vi "Stream LLP Packets to Disk.vi"(0 "fpga interface in":refnum<k20>, 1 "bytes acquired indicator ref":refnum<vi>, 5 "serial input channel":string, 7 "base packet file path":path, 9 "fetch size (elements)":u32=40960, 11 "error in (no error)":errorcluster, 12 "fetch timeout (s)":dbl=1.0, 13 "log to disk":bool=TRUE) -> (4 "fpga interface out":refnum<k20>, 6 "file path out":path, 8 "acquisition error":bool, 15 "error out":errorcluster)   [LabVIEW 2023, in "GettingStarted_Acq_148X_Host.lvlib"]
uses:
  GettingStarted_Acq_148X_Host.lvlib
  Types/148x_Acq_FPGA_Reference.ctl
  0829f115-c11d-4785-86b3-38f743f517d6.vi
  <vilib>/rvi/errors/niLvFpgaAdjustHostInterfaceError.vi
  <vilib>/rvi/interface/nirviMethod/nirviMethod.xnode
  <vilib>/rvi/interface/nirviReadWriteControl/nirviReadWriteControl.xnode
  <vilib>/FPGAPlugInAG/Dynamic/niLvFpga_AcquireReadRegionFifo_Dynamic.vi
  <vilib>/rvi/errors/niLvFpgaMergeErrorWithErrorCode.vi
  <instrlib>/FlexRIO/Automotive Vision Utility/v1/Host/Automotive Vision Utility.lvlib
  Common/GettingStarted_Common_148X_Host.lvlib
  NiFpgaLv.dll
  <vilib>/rvi/interface/Simulation/niFpgaSimulationCallBeginRW.vi
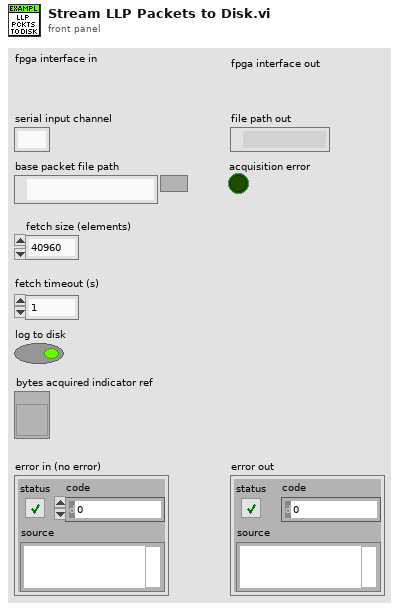
[diagram p1: front panel]
types:
  T1 = typedef "Automotive Vision Utility.lvlib/Serial Channel Type.ctl" = enum16{"Serial Input Channel", "Serial Output Channel", "Unknown Channel Type"}
  T2 = typedef "GettingStarted_Acq_148X_Host.lvlib/148x_Acq_FPGA_Reference.ctl" = refnum<k20>
  T3 = enum16{"open", "open or create", "create or replace", "create", "open (read-only)"}
  T4 = cluster{"acq state":enum8{"Idle", "Wait for First Packet Header", "Acquire", "Wait for Last Packet Header", "Wait for End of Last Packet"}, "stop timed out":bool, "bad packet header":bool, "bad packet payload":bool, "bad packet size":bool, "dram status":cluster{"bytes written":u64, "bytes read":u64, "overflow":bool, "partition full":bool, "last byte flushed":bool}}[]
  T5 = cluster{"acq state":enum8{"Idle", "Wait for First Packet Header", "Acquire", "Wait for Last Packet Header", "Wait for End of Last Packet"}, "stop timed out":bool, "bad packet header":bool, "bad packet payload":bool, "bad packet size":bool, "dram status":cluster{"bytes written":u64, "bytes read":u64, "overflow":bool, "partition full":bool, "last byte flushed":bool}}
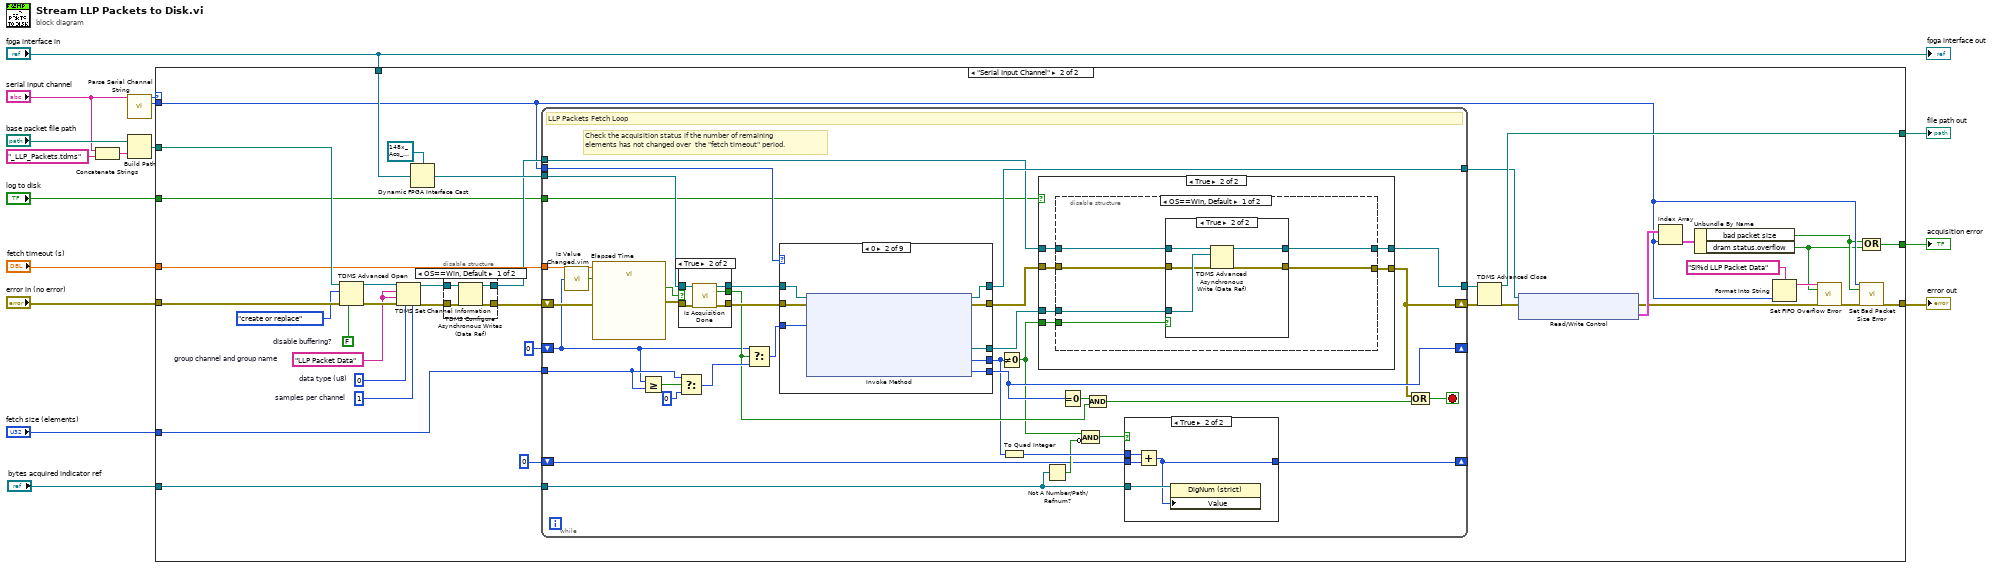
[diagram p0: block diagram]
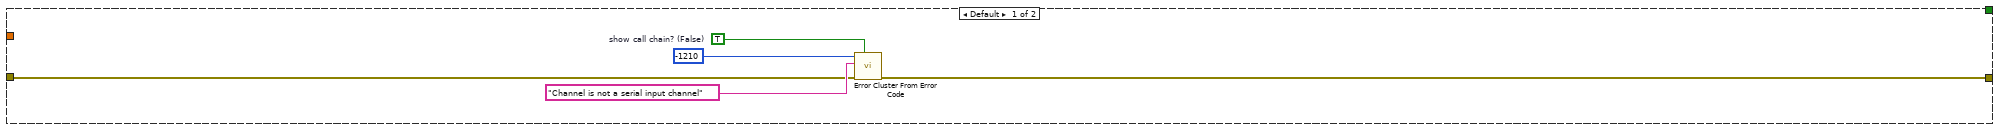
[diagram p2: hidden frame]
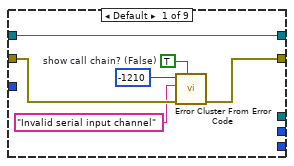
[diagram p6: hidden frame]
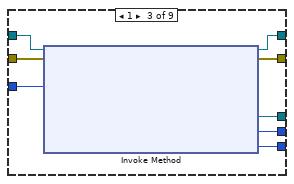
[diagram p7: hidden frame]
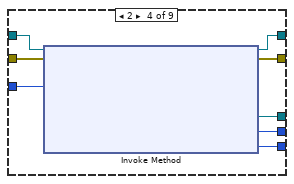
[diagram p8: hidden frame]
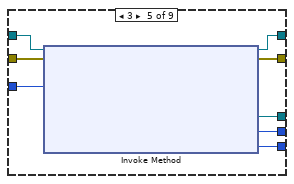
[diagram p9: hidden frame]
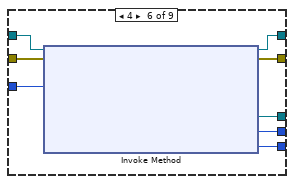
[diagram p10: hidden frame]
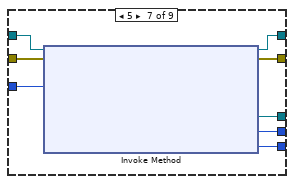
[diagram p11: hidden frame]
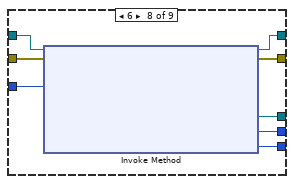
[diagram p12: hidden frame]
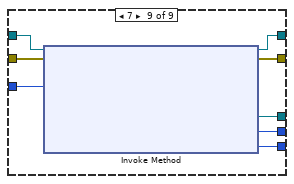
[diagram p13: hidden frame]
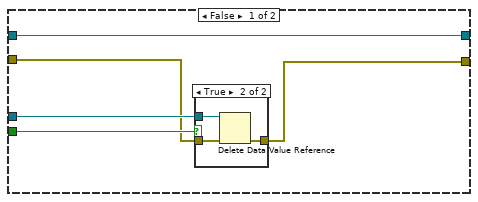
[diagram p14: hidden frame]
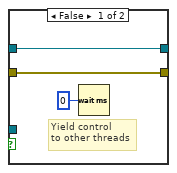
[diagram p16: hidden frame]
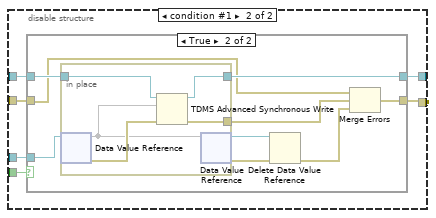
[diagram p17: hidden frame]
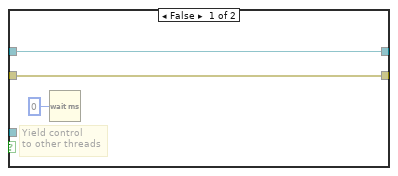
[diagram p18: hidden frame]
diagram:
  n1 = Concatenate Strings("serial input channel", "_LLP_Packets.tdms") -> (w9:string)
  n2 = call <instrlib>:"Parse Serial Channel String.vi"("serial channel string"="serial input channel") -> ("serial channel type"=w12:T1, "channel number"=w13:i32)  [unwired: 13 in]
  n3 = Build Path(base path="base packet file path", name or relative path=w9) -> (appended path=w6:path)
  n4 = case shown="\"Serial Input Channel\"" w12 {
    tunnel: "error in (no error)" -> [w18 w59]
    tunnel: w6 -> [_ w53]
    tunnel: [w17 w26] -> w15
    tunnel: [_ w22] -> w14
    tunnel: w13 -> [_ w25]
    tunnel: "fetch size (elements)" -> [_ w49]
    tunnel: "fpga interface in" -> [_ w48]
    tunnel: [_ w45] -> w5
    tunnel: "fetch timeout (s)" -> [_ w44]
    tunnel: "log to disk" -> [_ w30]
    tunnel: "bytes acquired indicator ref" -> [_ w28]
    frame Default {
      w19 = TRUE  # show call chain? (False)
      n5 = call <vilib>:"Error Cluster From Error Code.vi"("show call chain? (False)"=w19, "error in (no error)"=w18, "error message (\"\")"="Channel is not a serial input channel" ("error message (\"\")"), "error code (0)"=-1210) -> ("error out"=w17:errorcluster)  [unwired: 5 in]
    }
    frame "Serial Input Channel" {
      w55 = u32 1  # samples per channel
      w51 = FALSE  # disable buffering?
      w43 = u8 0  # data type (u8)
      w38 = "LLP Packet Data"  # group channel and group name
      n6 = TDMS Advanced Open(6:w51, 8:w59, 10:T3."create or replace" ("operation (0:open)"), 11:w53) -> (0:w39:errorcluster, 3:w57:refnum<k34>)  [unwired: 1 in, 1 out]
      n7 = TDMS Set Channel Information(4:w55, 6:w43, 8:w39, 9:w38, 10:w38, 11:w57) -> (0:w34:errorcluster, 3:w37:refnum<k34>)  [unwired: 1 in]
      n8 = Dynamic FPGA Interface Cast(Session In=T2 refnum ("FPGA VI Reference Out"), Type=w48) -> (Session Out=w46:T2)
      n9 = disable-structure shown="OS==Win, Default" {
        disable-tunnel: w34 -> [w60 w65]
        disable-tunnel: [w63 w64] -> w36
        disable-tunnel: [w62 w65] -> w35
        disable-tunnel: w37 -> [w61 w64]
        frame condition #0 (active) {
          n10 = TDMS Configure Asynchronous Writes (Data Ref)(8:w60, 11:w61) -> (0:w62:errorcluster, 3:w63:refnum<k34>)  [unwired: 2 in]
        }
        frame condition #1 {
        }
      }
      n11 = while {
        shift-right: [w78] -> w58
        shift-left: w35 -> [w84]
        tunnel: w46 -> [w88]
        shift-right: [w80] -> _
        shift-left: u32 0 ("Elements Remaining") -> [w81]
        tunnel: w36 -> [w77]
        tunnel: [w79] -> w54
        tunnel: [w96] -> w41
        tunnel: w25 -> [w99]
        tunnel: w49 -> [w90]
        tunnel: w44 -> [w95]
        tunnel: w30 -> [w74]
        shift-right: [w68] -> _
        shift-left: i64 0 -> [w67]
        tunnel: w28 -> [w69]
        stop <- w100 stop-if-true
        # "Check the acquisition status if the number of remaining \nelements has not changed over  the \"fetch timeout\" period."
        # "LLP Packets Fetch Loop"
        n12 = call "Is Value Changed.vim"("value"=w81) -> ("changed or first call?"=w94:bool)
        n13 = call "Elapsed Time"("Time Target (s)"=w95, "Reset"=w94, "error in (no error)"=w84) -> ("Time has Elapsed"=w86:bool, "error out"=w83:errorcluster)  [unwired: 9 in, 6 out]
        n14 = Greater Or Equal?(x=w81, y=w90) -> (x >= y?=w93:bool)
        n15 = case shown="True" w86 {
          tunnel: w83 -> [w107 w112]
          tunnel: [w107 w111] -> w89
          tunnel: w88 -> [w106 w110]
          tunnel: [w106 w109] -> w87
          tunnel: [_ w108] -> w85
          frame False {
          }
          frame True {
            n16 = call "Is Acquisition Done.vi"("fpga interface in"=w110, "error in (no error)"=w112) -> ("fpga interface out"=w109:T2, "acquisition done"=w108:bool, "error out"=w111:errorcluster)  [unwired: 11 in]
          }
        }
        n17 = Select(t=w90, s=w93, f=u32 0 ("Elements Remaining")) -> (s? t:f=w91:u32)
        n18 = Select(t=w81, s=w85, f=w91) -> (s? t:f=w92:u32)
        n19 = case shown="0" w99 {
          tunnel: w87 -> [w118 w126 w134 w142 w150 w158 w166 w174 w182]
          tunnel: w89 -> [w117 w125 w133 w141 w149 w157 w165 w173 w181]
          tunnel: [_ w124 w132 w140 w148 w156 w164 w172 w180] -> w75
          tunnel: [_ w123 w131 w139 w147 w155 w163 w171 w179] -> w66
          tunnel: w92 -> [_ w122 w130 w138 w146 w154 w162 w170 w178]
          tunnel: [w114 w120 w128 w136 w144 w152 w160 w168 w176] -> w76
          tunnel: [_ w121 w129 w137 w145 w153 w161 w169 w177] -> w80
          tunnel: [w118 w119 w127 w135 w143 w151 w159 w167 w175] -> w96
          frame Default {
            w113 = TRUE  # show call chain? (False)
            n20 = call <vilib>:"Error Cluster From Error Code.vi"("show call chain? (False)"=w113, "error in (no error)"=w117, "error message (\"\")"="Invalid serial input channel" ("error message (\"\")"), "error code (0)"=-1210) -> ("error out"=w114:errorcluster)  [unwired: 5 in]
          }
          frame 0 {
            n21 = xnode "Invoke Method"("FPGA VI Reference In"=w126, "error in"=w125, "Number of Elements"=w122) -> ("FPGA VI Reference Out"=w119:T2, "error out"=w120:errorcluster, "Read Region Reference"=w124:refnum<data-value>, "Elements In Region"=w123:u32, "Elements Remaining"=w121:u32)  [unwired: 1 in]
          }
          frame 1 {
            n22 = xnode "Invoke Method"("FPGA VI Reference In"=w134, "error in"=w133, "Number of Elements"=w130) -> ("FPGA VI Reference Out"=w127:T2, "error out"=w128:errorcluster, "Read Region Reference"=w132:refnum<data-value>, "Elements In Region"=w131:u32, "Elements Remaining"=w129:u32)  [unwired: 1 in]
          }
          frame 2 {
            n23 = xnode "Invoke Method"("FPGA VI Reference In"=w142, "error in"=w141, "Number of Elements"=w138) -> ("FPGA VI Reference Out"=w135:T2, "error out"=w136:errorcluster, "Read Region Reference"=w140:refnum<data-value>, "Elements In Region"=w139:u32, "Elements Remaining"=w137:u32)  [unwired: 1 in]
          }
          frame 3 {
            n24 = xnode "Invoke Method"("FPGA VI Reference In"=w150, "error in"=w149, "Number of Elements"=w146) -> ("FPGA VI Reference Out"=w143:T2, "error out"=w144:errorcluster, "Read Region Reference"=w148:refnum<data-value>, "Elements In Region"=w147:u32, "Elements Remaining"=w145:u32)  [unwired: 1 in]
          }
          frame 4 {
            n25 = xnode "Invoke Method"("FPGA VI Reference In"=w158, "error in"=w157, "Number of Elements"=w154) -> ("FPGA VI Reference Out"=w151:T2, "error out"=w152:errorcluster, "Read Region Reference"=w156:refnum<data-value>, "Elements In Region"=w155:u32, "Elements Remaining"=w153:u32)  [unwired: 1 in]
          }
          frame 5 {
            n26 = xnode "Invoke Method"("FPGA VI Reference In"=w166, "error in"=w165, "Number of Elements"=w162) -> ("FPGA VI Reference Out"=w159:T2, "error out"=w160:errorcluster, "Read Region Reference"=w164:refnum<data-value>, "Elements In Region"=w163:u32, "Elements Remaining"=w161:u32)  [unwired: 1 in]
          }
          frame 6 {
            n27 = xnode "Invoke Method"("FPGA VI Reference In"=w174, "error in"=w173, "Number of Elements"=w170) -> ("FPGA VI Reference Out"=w167:T2, "error out"=w168:errorcluster, "Read Region Reference"=w172:refnum<data-value>, "Elements In Region"=w171:u32, "Elements Remaining"=w169:u32)  [unwired: 1 in]
          }
          frame 7 {
            n28 = xnode "Invoke Method"("FPGA VI Reference In"=w182, "error in"=w181, "Number of Elements"=w178) -> ("FPGA VI Reference Out"=w175:T2, "error out"=w176:errorcluster, "Read Region Reference"=w180:refnum<data-value>, "Elements In Region"=w179:u32, "Elements Remaining"=w177:u32)  [unwired: 1 in]
          }
        }
        n29 = Not Equal To 0?(x=w66) -> (x != 0?=w70:bool)
        n30 = To Quad Integer(1:w66) -> (0:w73:i64)
        n31 = case shown="True" w74 {
          tunnel: w77 -> [w187 w197]
          tunnel: w76 -> [w184 w196]
          tunnel: w75 -> [w186 w195]
          tunnel: [w187 w194] -> w79
          tunnel: [w183 w193] -> w78
          tunnel: w70 -> [w185 w192]
          frame False {
            n32 = case shown="True" w185 {
              tunnel: w184 -> [w188 w191]
              tunnel: w186 -> [_ w190]
              tunnel: [w188 w189] -> w183
              frame False {
              }
              frame True {
                n33 = Delete Data Value Reference(data value reference=w190, error in=w191) -> (error out=w189:errorcluster)  [unwired: 1 out]
              }
            }
          }
          frame True {
            n34 = disable-structure shown="OS==Win, Default" {
              disable-tunnel: w197 -> [w201 w217]
              disable-tunnel: w196 -> [w200 w216]
              disable-tunnel: w195 -> [w199 w215]
              disable-tunnel: w192 -> [w198 w214]
              disable-tunnel: [w203 w213] -> w194
              disable-tunnel: [w202 w212] -> w193
              frame condition #0 (active) {
                n35 = case shown="True" w198 {
                  tunnel: w201 -> [w205 w211]
                  tunnel: [w205 w209] -> w203
                  tunnel: w200 -> [w204 w207]
                  tunnel: [w204 w208] -> w202
                  tunnel: w199 -> [_ w210]
                  frame False {
                    # "Yield control\nto other threads"
                    n36 = Wait (ms)(milliseconds to wait=u32 0) -> ()  [unwired: 1 out]
                  }
                  frame True {
                    n37 = TDMS Advanced Asynchronous Write (Data Ref)(8:w207, 10:w210, 11:w211) -> (0:w208:errorcluster, 3:w209:refnum<k34>)  [unwired: 1 in]
                  }
                }
              }
              frame condition #1 {
                n38 = case shown="True" w214 {
                  tunnel: w217 -> [w219 w228]
                  tunnel: [w219 w225] -> w213
                  tunnel: w216 -> [w218 w224]
                  tunnel: [w218 w221] -> w212
                  tunnel: w215 -> [_ w229]
                  frame False {
                    # "Yield control\nto other threads"
                    n39 = Wait (ms)(milliseconds to wait=u32 0) -> ()  [unwired: 1 out]
                  }
                  frame True {
                    n40 = in-place {
                      in-place-border: w228 -> [w234]
                      in-place-border: [w231] -> w223
                      in-place-border: [w230] -> w225
                      n41 = in-place-dvr #1(w229) -> (w232:u8[], w233:errorcluster)
                      n42 = TDMS Advanced Synchronous Write(8:w233, 10:w232, 11:w234) -> (0:w231:errorcluster, 3:w230:refnum<k34>)
                      n43 = in-place-dvr #1(w232) -> (w226:refnum<data-value>, w227:errorcluster)
                    }
                    n44 = Delete Data Value Reference(data value reference=w226, error in=w227) -> (error out=w222:errorcluster)  [unwired: 1 out]
                    n45 = Merge Errors(w224, w223, w222) -> (w221:errorcluster)
                  }
                }
              }
            }
          }
        }
        n46 = Not A Number/Path/Refnum?(number/path/refnum=w69) -> (NaN/Path/Refnum?=w71:bool)
        n47 = Equal To 0?(x=w80) -> (x = 0?=w82:bool)
        n48 = Compound Arithmetic op=AND(w70, invert w71) -> (w72:bool)
        n49 = Compound Arithmetic op=AND(w82, w85) -> (w97:bool)
        n50 = case shown="True" w72 {
          tunnel: w67 -> [w101 w105]
          tunnel: w73 -> [_ w104]
          tunnel: [w101 w102] -> w68
          tunnel: w69 -> [_ w103]
          frame False {
          }
          frame True {
            n51 = Add(x=w104, y=w105) -> (x+y=w102:i64)
            n52 = property class="DigNum (strict)"(reference=w103, "Value"=w102) -> ()  [unwired: 1 in, 2 out]
          }
        }
        n53 = Compound Arithmetic op=OR(w78, w97) -> (w100:bool)
      }
      n54 = TDMS Advanced Close(8:w58, 11:w54) -> (0:w42:errorcluster, 3:w45:path)  [unwired: 2 in]
      n55 = xnode "Read/Write Control"("FPGA VI Reference In"=w41, "error in"=w42) -> ("error out"=w33:errorcluster, "serial input channel status"=w40:T4)  [unwired: 1 out]
      n56 = Index Array(array=w40, index=w25) -> (element=w50:T5)
      n57 = Unbundle By Name(w50) -> ("bad packet size"=w24:bool, "dram status.overflow"=w23:bool)
      n58 = Format Into String(format string="SI%d LLP Packet Data" ("fifo name"), w25) -> (resulting string=w32:string)  [unwired: 2 in, 1 out]
      n59 = call "Set FIFO Overflow Error.vi"("fifo name"=w32, "overflow"=w23, "error in (no error)"=w33) -> ("error out"=w27:errorcluster)  [unwired: 12 in]
      n60 = call "Set Bad Packet Size Error.vi"("serial input channel"=w25, "bad packet size"=w24, "error in (no error)"=w27) -> ("error out"=w26:errorcluster)  [unwired: 12 in]
      n61 = Compound Arithmetic op=OR(w24, w23) -> (w22:bool)
    }
  }
  "error out" <- w15
  "acquisition error" <- w14
  "file path out" <- w5
  "fpga interface out" <- "fpga interface in"
